vi "RemoteVI Loop Init.vi"(0 "VI":refnum<vi>, 5 "share":T3, 7 "port":u16=8088, 9 "fps":dbl=20.0, 11 "error in":errorcluster) -> (4 "context":T2, 6 "state":T1, 15 "error out":errorcluster)   [LabVIEW 2020, in "RemoteVI.lvlib"]
doc: "Before the server loop starts: RemoteVI Server Setup.vi prepares the page, the greeting, the geometry and the target (a VI's panel, or a window - over VI Server when its LabVIEW runs one, else Win32 only). Returns the context (what does not change while the share runs, with the share's entry for the status: kind VI for a VI's panel, VI Server for a window of another LabVIEW reached over VI Server, Window for a window shared through Win32 only, and when the share started) and the initial loop state."
uses:
  RemoteVI.lvlib
panel:
  in  "no state yet":T1
  in  "no context yet":T2
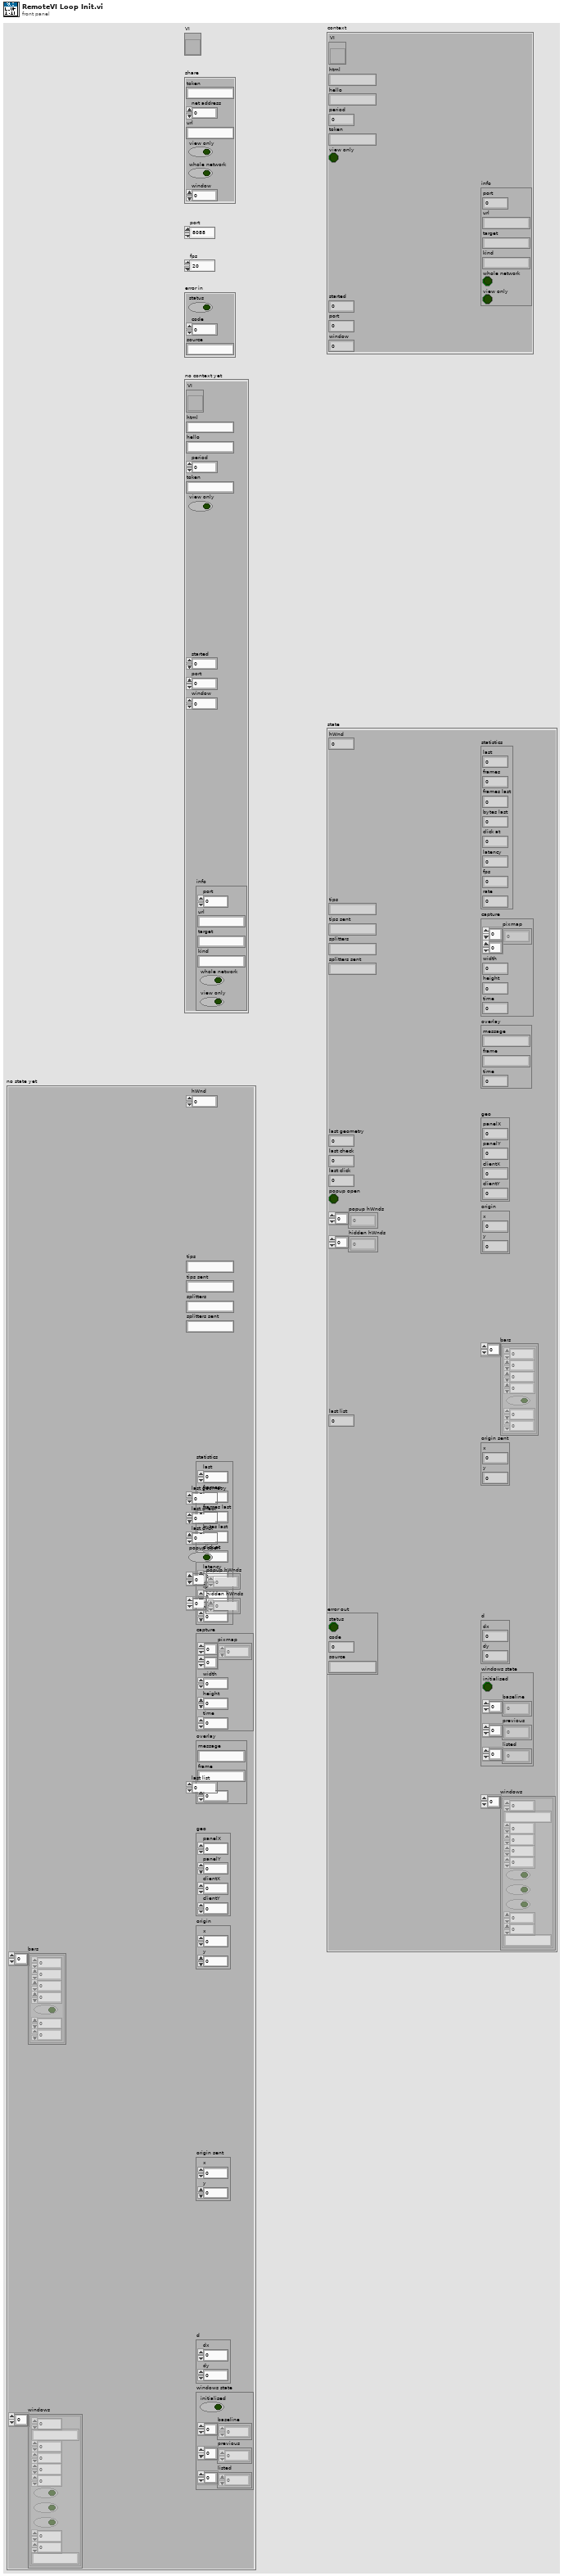
[diagram p1: front panel]
types:
  T1 = cluster{"statistics":cluster{"last":dbl, "frames":u32, "frames last":u32, "bytes last":dbl, "click at":dbl, "latency":dbl, "fps":dbl, "rate":dbl}, "capture":cluster{"pixmap":u32[][], "width":i32, "height":i32, "time":u32}, "overlay":cluster{"message":string, "frame":string, "time":u32}, "hWnd":u64, "geo":cluster{"panelX":i32, "panelY":i32, "clientX":i32, "clientY":i32}, "origin":cluster{"x":i32, "y":i32}, "tips":string, "tips sent":string, "splitters":string, "splitters sent":string, "bars":cluster{"x":i32, "y":i32, "w":i32, "h":i32, "vertical":bool, "min":i32, "max":i32}[], "origin sent":cluster{"x":i32, "y":i32}, "last geometry":u32, "last check":u32, "last click":u32, "popup open":bool, "popup hWnds":u64[], "hidden hWnds":u64[], "d":cluster{"dx":i32, "dy":i32}, "windows state":cluster{"initialised":bool, "baseline":u64[], "previous":u64[], "listed":u64[]}, "last list":u32, "windows":cluster{"id":u64, "title":string, "x":i32, "y":i32, "w":i32, "h":i32, "modal":bool, "active":bool, "closable":bool, "sx":i32, "sy":i32, "class":string}[]}
  T2 = cluster{"VI":refnum<vi>, "html":string, "hello":string, "period":dbl, "token":string, "view only":bool, "info":cluster{"port":u16, "url":string, "target":string, "kind":string, "whole network":bool, "view only":bool}, "started":dbl, "port":u16, "window":u64}
  T3 = cluster{"token":string, "net address":u32, "url":string, "view only":bool, "whole network":bool, "window":u64}
  T4 = cluster{"port":u16, "url":string, "target":string, "kind":string, "whole network":bool, "view only":bool}
  T5 = cluster{"panelX":i32, "panelY":i32, "clientX":i32, "clientY":i32}
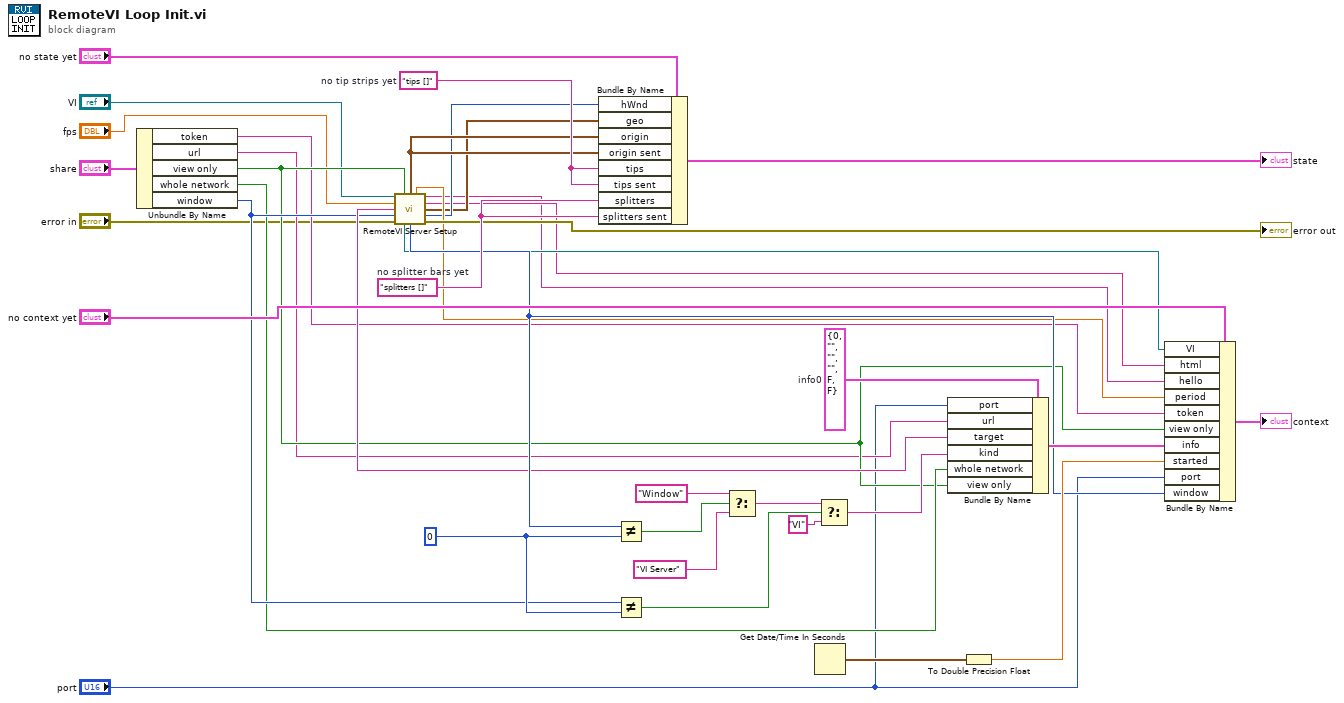
[diagram p0: block diagram]
diagram:
  w37 = "splitters []"  # no splitter bars yet
  w36 = "tips []"  # no tip strips yet
  w29 = T4 {"port"=0, "url"="", "target"="", "kind"="", "whole network"=FALSE, "view only"=FALSE}  # info0
  w21 = u64 0
  n1 = Unbundle By Name("share") -> ("token"=w6:string, "url"=w7:string, "view only"=w8:bool, "whole network"=w9:bool, "window"=w10:u64)
  n2 = call "RemoteVI Server Setup.vi"("VI"="VI", "view only?"=w8, "fps"="fps", "window"=w10, "error in"="error in") -> ("origin"=w15:cluster{"x":i32, "y":i32}, "period"=w16:dbl, "hello"=w11:string, "html"=w12:string, "VI name"=w17:string, "geo"=w13:T5, "hWnd"=w14:u64, "VI out"=w19:refnum<vi>, "window out"=w20:u64, "error out"=→"error out":errorcluster)  [unwired: 1 out]
  n3 = Bundle By Name(cluster="no state yet", "hWnd"=w14, "geo"=w13, "origin"=w15, "origin sent"=w15, "tips"=w36, "tips sent"=w36, "splitters"=w37, "splitters sent"=w37) -> (→"state":T1)
  n4 = Not Equal?(x=w20, y=w21) -> (x != y?=w23:bool)
  n5 = Not Equal?(x=w10, y=w21) -> (x != y?=w22:bool)
  n6 = Select(t="Window", s=w23, f="VI Server") -> (s? t:f=w27:string)
  n7 = Get Date/Time In Seconds() -> (seconds since 1Jan1904=w31:timestamp)
  n8 = Select(t=w27, s=w22, f="VI") -> (s? t:f=w28:string)
  n9 = Bundle By Name(cluster=w29, "port"="port", "url"=w7, "target"=w17, "kind"=w28, "whole network"=w9, "view only"=w8) -> (w30:T4)
  n10 = To Double Precision Float(number=w31) -> (double precision float=w32:dbl)
  n11 = Bundle By Name(cluster="no context yet", "VI"=w19, "html"=w12, "hello"=w11, "period"=w16, "token"=w6, "view only"=w8, "info"=w30, "started"=w32, "port"="port", "window"=w20) -> (→"context":T2)
